vi "VIH HelpGen - Image - Convert Image to Image.vi"(8 "BG Color (white)":u32(colorbox)=16777215, 9 "color depth (as source)":i32=24, 11 "image data":T1) -> (3 "image data out":T1)   [LabVIEW 2014]
doc: "::: VI Helpeks :::\nCopyright (c) 2000-2026 Konstantin Shifershteyn. All rights reserved."
uses:
  <vilib>/picture/picture.llb/imagedata.ctl
panel:
  # "VI Helpeks\nCopyright (c) 2012-2026 Konstantin Shifershteyn"
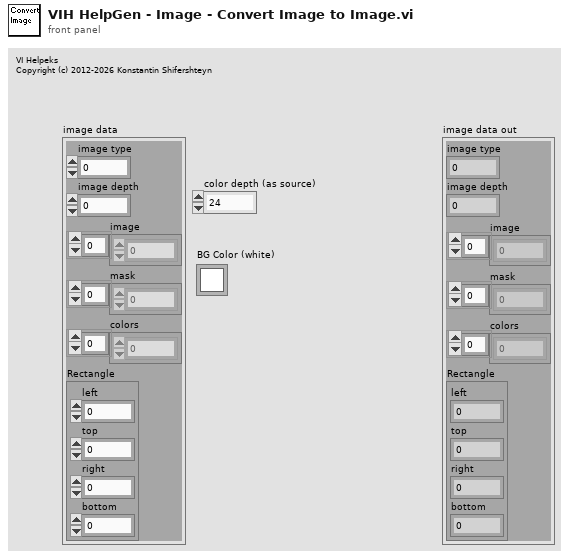
[diagram p1: front panel]
types:
  T1 = typedef "imagedata.ctl" = cluster{"image type":i32, "image depth":i32, "image":u8[], "mask":u8[], "colors":u32[], "Rectangle":cluster{"left":i16, "top":i16, "right":i16, "bottom":i16}}
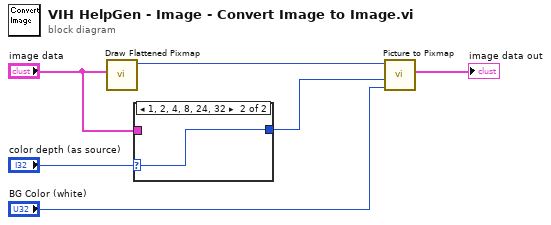
[diagram p0: block diagram]
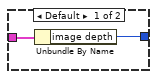
[diagram p2: hidden frame]
diagram:
  n1 = call <vilib>:"Draw Flattened Pixmap.vi"("image data"="image data") -> ("new picture"=w6:picture)  [unwired: 8 in]
  n2 = case shown="1, 2, 4, 8, 24, 32" "color depth (as source)" {
    selector: "color depth (as source)" -> [_ w9]
    tunnel: "image data" -> [w8 _]
    tunnel: [w7 w9] -> w1
    frame Default {
      n3 = Unbundle By Name(w8) -> ("image depth"=w7:i32)
    }
    frame 1, 2, 4, 8, 24, 32 {
    }
  }
  n4 = call <vilib>:"Picture to Pixmap.vi"("Background Color"="BG Color (white)", "depth"=w1, "picture"=w6) -> ("image data"=→"image data out":T1)  [unwired: 7 in, 1 out]
